vi "Grab Server Values.vi"(6 "error in (no error)":errorcluster, 8 "Lines":T1[](array[typedef]) {"OPC UA Data Type" items=["Boolean"=1, "SByte"=2, "Byte"=3, "Int16"=4, "UInt16"=5, "Int32"=6, "UInt32"=7, "Int64"=8, "UInt64"=9, "Float"=10, "Double"=11, "String"=12, "DateTime"=13, "ByteString"=15, "Array of Boolean"=101, "Array of SByte"=102, "Array of Byte"=103, "Array of Int16"=104, "Array of UInt16"=105, "Array of Int32"=106, "Array of UInt32"=107, "Array of Int64"=108, "Array of UInt64"=109, "Array of Float"=110, "Array of Double"=111, "Array of String"=112, "Array of DateTime"=113, "Array of ByteString"=115]}, 9 "OPC UA server refnum":refnum<k21>) -> (0 "error out":errorcluster, 2 "Server Data":T3(array[cluster]), 3 "OPC UA server refnum":refnum<k21>)   [LabVIEW 2014, in "OPC UA Client Tests.lvlib"]
doc: "Poll every node of an OPC server defined in Lines input and pass its data out as a flattened string"
uses:
  OPC UA Client Tests.lvlib
  module/configuration/Line.ctl
  <vilib>/NI/Tag Bus Module Framework/channel/TBM channel.lvclass
  module/configuration/OPC UA Data Type.ctl
  <vilib>/OPCUA/server/Read Bool.vi
  <vilib>/OPCUA/server/Read SByte.vi
  <vilib>/OPCUA/server/Read Byte.vi
  <vilib>/OPCUA/server/Read Int16.vi
  <vilib>/OPCUA/server/Read UInt16.vi
  <vilib>/OPCUA/server/Read Int32.vi
  <vilib>/OPCUA/server/Read UInt32.vi
  <vilib>/OPCUA/server/Read Int64.vi
  <vilib>/OPCUA/server/Read UInt64.vi
  <vilib>/OPCUA/server/Read Float.vi
  <vilib>/OPCUA/server/Read Double.vi
  <vilib>/OPCUA/server/Read String.vi
  <vilib>/OPCUA/server/Read Date Time.vi
  <vilib>/OPCUA/server/Read Byte String.vi
  <vilib>/OPCUA/server/Read Bool Array.vi
  <vilib>/OPCUA/server/Read SByte Array.vi
  <vilib>/OPCUA/server/Read Byte Array.vi
  <vilib>/OPCUA/server/Read Int16 Array.vi
  <vilib>/OPCUA/server/Read UInt16 Array.vi
  <vilib>/OPCUA/server/Read Int32 Array.vi
  <vilib>/OPCUA/server/Read UInt32 Array.vi
  <vilib>/OPCUA/server/Read Int64 Array.vi
  <vilib>/OPCUA/server/Read UInt64 Array.vi
  <vilib>/OPCUA/server/Read Float Array.vi
  <vilib>/OPCUA/server/Read Double Array.vi
  <vilib>/OPCUA/server/Read String Array.vi
  <vilib>/OPCUA/server/Read Date Time Array.vi
  <vilib>/OPCUA/server/Read Byte String Array.vi
  <vilib>/opcua/NI OPC UA Server.lvlib
  module/configuration/OPC UA Client configuration.lvclass
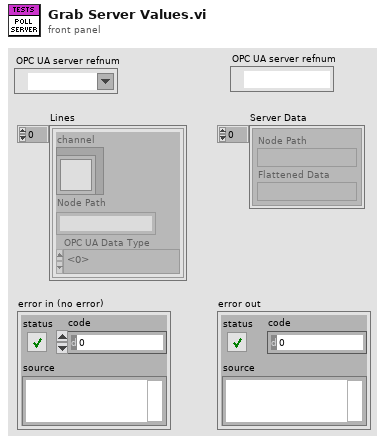
[diagram p1: front panel]
types:
  T1 = typedef "OPC UA Client configuration.lvclass/Line.ctl" = cluster{"channel":refnum<class "TBM channel.lvclass">, "Node Path":string, "OPC UA Data Type":T2}
  T2 = typedef "OPC UA Client configuration.lvclass/OPC UA Data Type.ctl" = u16
  T3 = cluster{"Node Path":string, "Flattened Data":string}[]
  T4 = cluster{"Node Path":string, "Flattened Data":string}
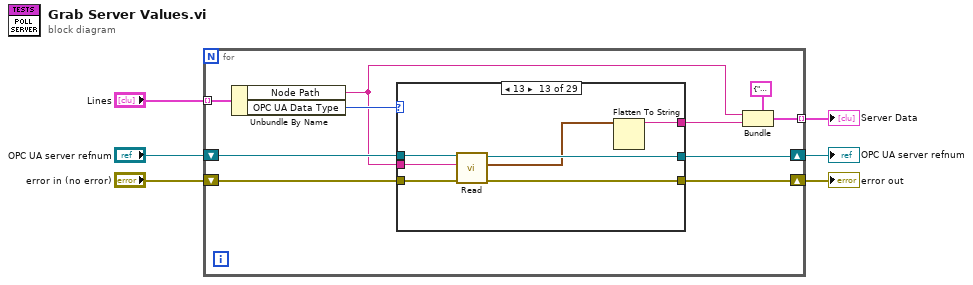
[diagram p0: block diagram]
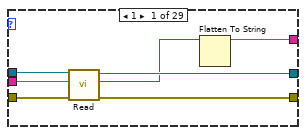
[diagram p2: hidden frame]
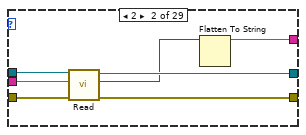
[diagram p3: hidden frame]
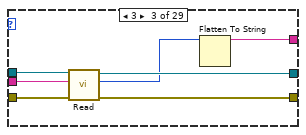
[diagram p4: hidden frame]
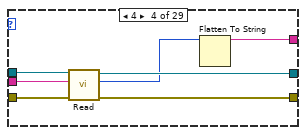
[diagram p5: hidden frame]
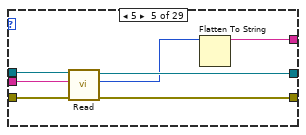
[diagram p6: hidden frame]
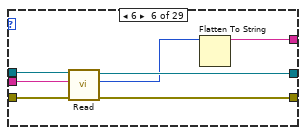
[diagram p7: hidden frame]
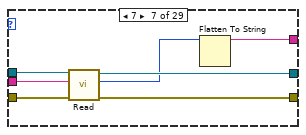
[diagram p8: hidden frame]
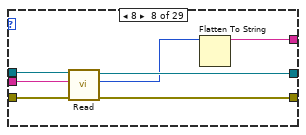
[diagram p9: hidden frame]
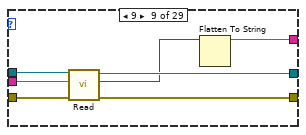
[diagram p10: hidden frame]
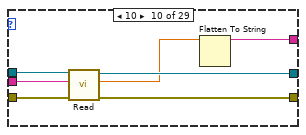
[diagram p11: hidden frame]
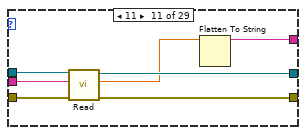
[diagram p12: hidden frame]
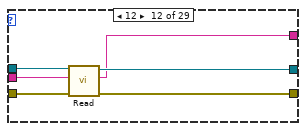
[diagram p13: hidden frame]
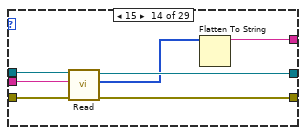
[diagram p14: hidden frame]
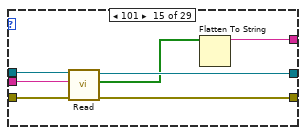
[diagram p15: hidden frame]
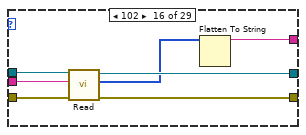
[diagram p16: hidden frame]
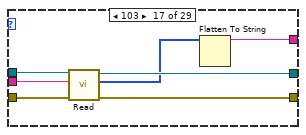
[diagram p17: hidden frame]
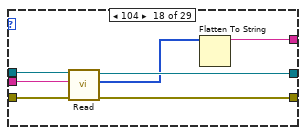
[diagram p18: hidden frame]
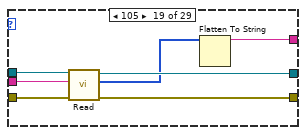
[diagram p19: hidden frame]
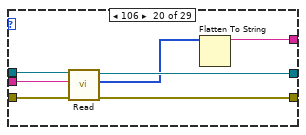
[diagram p20: hidden frame]
diagram:
  n1 = for {
    shift-right: [w10] -> w5
    shift-left: "OPC UA server refnum" -> [w12]
    tunnel: "Lines" -> [w16] mode=indexing
    shift-right: [w7] -> w2
    shift-left: "error in (no error)" -> [w8]
    tunnel: [w13] -> w1 mode=indexing
    n2 = Unbundle By Name(w16) -> ("Node Path"=w11:string, "OPC UA Data Type"=w15:T2)
    n3 = case shown="13" w15 {
      tunnel: w12 -> [w23 w30 w37 w44 w51 w58 w65 w72 w79 w86 w93 w99 w106 w113 w120 w127 w134 w141 w148 w155 w162 w169 w176 w183 w190 w197 w204 w211 w213]
      tunnel: w11 -> [w22 w29 w36 w43 w50 w57 w64 w71 w78 w85 w92 w98 w105 w112 w119 w126 w133 w140 w147 w154 w161 w168 w175 w182 w189 w196 w203 w210 _]
      tunnel: [w21 w28 w35 w42 w49 w56 w63 w70 w77 w84 w91 w97 w104 w111 w118 w125 w132 w139 w146 w153 w160 w167 w174 w181 w188 w195 w202 w209 w213] -> w10
      tunnel: [w19 w26 w33 w40 w47 w54 w61 w68 w75 w82 w89 w96 w100 w109 w116 w123 w130 w137 w144 w151 w158 w165 w172 w179 w186 w193 w200 w207 "" ("data string")] -> w9
      tunnel: w8 -> [w18 w25 w32 w39 w46 w53 w60 w67 w74 w81 w88 w95 w103 w108 w115 w122 w129 w136 w143 w150 w157 w164 w171 w178 w185 w192 w199 w206 w214]
      tunnel: [w17 w24 w31 w38 w45 w52 w59 w66 w73 w80 w87 w94 w102 w107 w114 w121 w128 w135 w142 w149 w156 w163 w170 w177 w184 w191 w198 w205 w214] -> w7
      frame 1 {
        n4 = call-poly <vilib>:"Read.vi"("error in (no error)"=w18, "node path"=w22, "OPC UA server refnum in"=w23) -> ("error out"=w17:errorcluster, "value"=w20:bool, "OPC UA server refnum out"=w21:refnum<k21>)  [unwired: 4 in, 2 out]
        n5 = Flatten To String(anything=w20) -> (data string=w19:string)  [unwired: 3 in, 2 out]
      }
      frame 2 {
        n6 = call-poly <vilib>:"Read.vi"("error in (no error)"=w25, "node path"=w29, "OPC UA server refnum in"=w30) -> ("error out"=w24:errorcluster, "value"=w27:i8, "OPC UA server refnum out"=w28:refnum<k21>)  [unwired: 4 in, 2 out]
        n7 = Flatten To String(anything=w27) -> (data string=w26:string)  [unwired: 3 in, 2 out]
      }
      frame 3 {
        n8 = call-poly <vilib>:"Read.vi"("error in (no error)"=w32, "node path"=w36, "OPC UA server refnum in"=w37) -> ("error out"=w31:errorcluster, "value"=w34:u8, "OPC UA server refnum out"=w35:refnum<k21>)  [unwired: 4 in, 2 out]
        n9 = Flatten To String(anything=w34) -> (data string=w33:string)  [unwired: 3 in, 2 out]
      }
      frame 4 {
        n10 = call-poly <vilib>:"Read.vi"("error in (no error)"=w39, "node path"=w43, "OPC UA server refnum in"=w44) -> ("error out"=w38:errorcluster, "value"=w41:i16, "OPC UA server refnum out"=w42:refnum<k21>)  [unwired: 4 in, 2 out]
        n11 = Flatten To String(anything=w41) -> (data string=w40:string)  [unwired: 3 in, 2 out]
      }
      frame 5 {
        n12 = call-poly <vilib>:"Read.vi"("error in (no error)"=w46, "node path"=w50, "OPC UA server refnum in"=w51) -> ("error out"=w45:errorcluster, "value"=w48:u16, "OPC UA server refnum out"=w49:refnum<k21>)  [unwired: 4 in, 2 out]
        n13 = Flatten To String(anything=w48) -> (data string=w47:string)  [unwired: 3 in, 2 out]
      }
      frame 6 {
        n14 = call-poly <vilib>:"Read.vi"("error in (no error)"=w53, "node path"=w57, "OPC UA server refnum in"=w58) -> ("error out"=w52:errorcluster, "value"=w55:i32, "OPC UA server refnum out"=w56:refnum<k21>)  [unwired: 4 in, 2 out]
        n15 = Flatten To String(anything=w55) -> (data string=w54:string)  [unwired: 3 in, 2 out]
      }
      frame 7 {
        n16 = call-poly <vilib>:"Read.vi"("error in (no error)"=w60, "node path"=w64, "OPC UA server refnum in"=w65) -> ("error out"=w59:errorcluster, "value"=w62:u32, "OPC UA server refnum out"=w63:refnum<k21>)  [unwired: 4 in, 2 out]
        n17 = Flatten To String(anything=w62) -> (data string=w61:string)  [unwired: 3 in, 2 out]
      }
      frame 8 {
        n18 = call-poly <vilib>:"Read.vi"("error in (no error)"=w67, "node path"=w71, "OPC UA server refnum in"=w72) -> ("error out"=w66:errorcluster, "value"=w69:i64, "OPC UA server refnum out"=w70:refnum<k21>)  [unwired: 4 in, 2 out]
        n19 = Flatten To String(anything=w69) -> (data string=w68:string)  [unwired: 3 in, 2 out]
      }
      frame 9 {
        n20 = call-poly <vilib>:"Read.vi"("error in (no error)"=w74, "node path"=w78, "OPC UA server refnum in"=w79) -> ("error out"=w73:errorcluster, "value"=w76:u64, "OPC UA server refnum out"=w77:refnum<k21>)  [unwired: 4 in, 2 out]
        n21 = Flatten To String(anything=w76) -> (data string=w75:string)  [unwired: 3 in, 2 out]
      }
      frame 10 {
        n22 = call-poly <vilib>:"Read.vi"("error in (no error)"=w81, "node path"=w85, "OPC UA server refnum in"=w86) -> ("error out"=w80:errorcluster, "value"=w83:sgl, "OPC UA server refnum out"=w84:refnum<k21>)  [unwired: 4 in, 2 out]
        n23 = Flatten To String(anything=w83) -> (data string=w82:string)  [unwired: 3 in, 2 out]
      }
      frame 11 {
        n24 = call-poly <vilib>:"Read.vi"("error in (no error)"=w88, "node path"=w92, "OPC UA server refnum in"=w93) -> ("error out"=w87:errorcluster, "value"=w90:dbl, "OPC UA server refnum out"=w91:refnum<k21>)  [unwired: 4 in, 2 out]
        n25 = Flatten To String(anything=w90) -> (data string=w89:string)  [unwired: 3 in, 2 out]
      }
      frame 12 {
        n26 = call-poly <vilib>:"Read.vi"("error in (no error)"=w95, "node path"=w98, "OPC UA server refnum in"=w99) -> ("error out"=w94:errorcluster, "value"=w96:string, "OPC UA server refnum out"=w97:refnum<k21>)  [unwired: 4 in, 2 out]
      }
      frame 13 {
        n27 = call-poly <vilib>:"Read.vi"("error in (error in)"=w103, "node path"=w105, "OPC UA server refnum in"=w106) -> ("error out"=w102:errorcluster, "value"=w101:timestamp, "OPC UA server refnum out"=w104:refnum<k21>)  [unwired: 4 in, 2 out]
        n28 = Flatten To String(anything=w101) -> (data string=w100:string)  [unwired: 3 in, 2 out]
      }
      frame 15 {
        n29 = call-poly <vilib>:"Read.vi"("error in (no error)"=w108, "node path"=w112, "OPC UA server refnum in"=w113) -> ("error out"=w107:errorcluster, "value"=w110:u8[], "OPC UA server refnum out"=w111:refnum<k21>)  [unwired: 4 in, 2 out]
        n30 = Flatten To String(anything=w110) -> (data string=w109:string)  [unwired: 3 in, 2 out]
      }
      frame 101 {
        n31 = call-poly <vilib>:"Read.vi"("error in (no error)"=w115, "node path"=w119, "OPC UA server refnum in"=w120) -> ("error out"=w114:errorcluster, "value"=w117:bool[], "OPC UA server refnum out"=w118:refnum<k21>)  [unwired: 4 in, 2 out]
        n32 = Flatten To String(anything=w117) -> (data string=w116:string)  [unwired: 3 in, 2 out]
      }
      frame 102 {
        n33 = call-poly <vilib>:"Read.vi"("error in (no error)"=w122, "node path"=w126, "OPC UA server refnum in"=w127) -> ("error out"=w121:errorcluster, "value"=w124:i8[], "OPC UA server refnum out"=w125:refnum<k21>)  [unwired: 4 in, 2 out]
        n34 = Flatten To String(anything=w124) -> (data string=w123:string)  [unwired: 3 in, 2 out]
      }
      frame 103 {
        n35 = call-poly <vilib>:"Read.vi"("error in (no error)"=w129, "node path"=w133, "OPC UA server refnum in"=w134) -> ("error out"=w128:errorcluster, "value"=w131:u8[], "OPC UA server refnum out"=w132:refnum<k21>)  [unwired: 4 in, 2 out]
        n36 = Flatten To String(anything=w131) -> (data string=w130:string)  [unwired: 3 in, 2 out]
      }
      frame 104 {
        n37 = call-poly <vilib>:"Read.vi"("error in (no error)"=w136, "node path"=w140, "OPC UA server refnum in"=w141) -> ("error out"=w135:errorcluster, "value"=w138:i16[], "OPC UA server refnum out"=w139:refnum<k21>)  [unwired: 4 in, 2 out]
        n38 = Flatten To String(anything=w138) -> (data string=w137:string)  [unwired: 3 in, 2 out]
      }
      frame 105 {
        n39 = call-poly <vilib>:"Read.vi"("error in (no error)"=w143, "node path"=w147, "OPC UA server refnum in"=w148) -> ("error out"=w142:errorcluster, "value"=w145:u16[], "OPC UA server refnum out"=w146:refnum<k21>)  [unwired: 4 in, 2 out]
        n40 = Flatten To String(anything=w145) -> (data string=w144:string)  [unwired: 3 in, 2 out]
      }
      frame 106 {
        n41 = call-poly <vilib>:"Read.vi"("error in (no error)"=w150, "node path"=w154, "OPC UA server refnum in"=w155) -> ("error out"=w149:errorcluster, "value"=w152:i32[], "OPC UA server refnum out"=w153:refnum<k21>)  [unwired: 4 in, 2 out]
        n42 = Flatten To String(anything=w152) -> (data string=w151:string)  [unwired: 3 in, 2 out]
      }
      frame 107 {
        n43 = call-poly <vilib>:"Read.vi"("error in (no error)"=w157, "node path"=w161, "OPC UA server refnum in"=w162) -> ("error out"=w156:errorcluster, "value"=w159:u32[], "OPC UA server refnum out"=w160:refnum<k21>)  [unwired: 4 in, 2 out]
        n44 = Flatten To String(anything=w159) -> (data string=w158:string)  [unwired: 3 in, 2 out]
      }
      frame 108 {
        n45 = call-poly <vilib>:"Read.vi"("error in (no error)"=w164, "node path"=w168, "OPC UA server refnum in"=w169) -> ("error out"=w163:errorcluster, "value"=w166:i64[], "OPC UA server refnum out"=w167:refnum<k21>)  [unwired: 4 in, 2 out]
        n46 = Flatten To String(anything=w166) -> (data string=w165:string)  [unwired: 3 in, 2 out]
      }
      frame 109 {
        n47 = call-poly <vilib>:"Read.vi"("error in (no error)"=w171, "node path"=w175, "OPC UA server refnum in"=w176) -> ("error out"=w170:errorcluster, "value"=w173:u64[], "OPC UA server refnum out"=w174:refnum<k21>)  [unwired: 4 in, 2 out]
        n48 = Flatten To String(anything=w173) -> (data string=w172:string)  [unwired: 3 in, 2 out]
      }
      frame 110 {
        n49 = call-poly <vilib>:"Read.vi"("error in (no error)"=w178, "node path"=w182, "OPC UA server refnum in"=w183) -> ("error out"=w177:errorcluster, "value"=w180:sgl[], "OPC UA server refnum out"=w181:refnum<k21>)  [unwired: 4 in, 2 out]
        n50 = Flatten To String(anything=w180) -> (data string=w179:string)  [unwired: 3 in, 2 out]
      }
      frame 111 {
        n51 = call-poly <vilib>:"Read.vi"("error in (no error)"=w185, "node path"=w189, "OPC UA server refnum in"=w190) -> ("error out"=w184:errorcluster, "value"=w187:dbl[], "OPC UA server refnum out"=w188:refnum<k21>)  [unwired: 4 in, 2 out]
        n52 = Flatten To String(anything=w187) -> (data string=w186:string)  [unwired: 3 in, 2 out]
      }
      frame 112 {
        n53 = call-poly <vilib>:"Read.vi"("error in (no error)"=w192, "node path"=w196, "OPC UA server refnum in"=w197) -> ("error out"=w191:errorcluster, "value"=w194:string[], "OPC UA server refnum out"=w195:refnum<k21>)  [unwired: 4 in, 2 out]
        n54 = Flatten To String(anything=w194) -> (data string=w193:string)  [unwired: 3 in, 2 out]
      }
      frame 113 {
        n55 = call-poly <vilib>:"Read.vi"("error in (no error)"=w199, "node path"=w203, "OPC UA server refnum in"=w204) -> ("error out"=w198:errorcluster, "value"=w201:timestamp[], "OPC UA server refnum out"=w202:refnum<k21>)  [unwired: 4 in, 2 out]
        n56 = Flatten To String(anything=w201) -> (data string=w200:string)  [unwired: 3 in, 2 out]
      }
      frame 115 {
        n57 = call-poly <vilib>:"Read.vi"("error in (no error)"=w206, "node path"=w210, "OPC UA server refnum in"=w211) -> ("error out"=w205:errorcluster, "value"=w208:u8[][], "OPC UA server refnum out"=w209:refnum<k21>)  [unwired: 4 in, 2 out]
        n58 = Flatten To String(anything=w208) -> (data string=w207:string)  [unwired: 3 in, 2 out]
      }
      frame 0, Default {
      }
    }
    n59 = Bundle(cluster=T4 {"Node Path"="", "Flattened Data"=""}, "Node Path"=w11, "Flattened Data"=w9) -> (w13:T4)
  }
  "Server Data" <- w1
  "error out" <- w2
  "OPC UA server refnum" <- w5
